vi "FuncVI-FileMove.vi"(5 "InstanceRef":T2, 9 "arg list":T1[](array[typedef]) {"num" format="%.2f"}) -> (0 "error out":bool, 3 "result":T1 {"num" format="%.2f"})   [LabVIEW 2021]
doc: "::: CalcExpress Toolkit :::\nCopyright (c) 2000-2026 Konstantin Shifershteyn. All rights reserved."
uses:
  cetypes.llb/CalcExpress Function Argument Info.ctl
  cetypes.llb/CalcExpress Instance RefNum.ctl
panel:
  in  "max arg num":i32=2
  in  "min arg num":i32=2
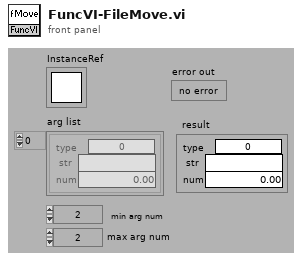
[diagram p1: front panel]
types:
  T1 = typedef "CalcExpress Function Argument Info.ctl" = cluster{"type":u32, "str":string, "num":dbl}
  T2 = typedef "CalcExpress Instance RefNum.ctl" = refnum<k1>
  T3 = enum32{"String", "DBL Number", "identifier", "1D Array of DBL", "2D Array of DBL", "CDB Number", "1D Array of CDB", "2D Array of CDB", "1D Array of String", "2D Array of String", "Unknown data type"}
  T4 = enum32{"existing file", "new file", "new or existing file", "existing dir", "new dir", "new or existing dir", "existing file (use LLBs)", "new file (use LLBs)", "new or existing file (use LLBs)", "new or existing file or directory (use LLBs)", "existing dir (use LLBs)", "new dir (use LLBs)", "new or existing dir (use LLBs)", "existing file or dir", "new file or dir", "new or existing file or dir", "existing file or dir (use LLBs)", "new file or dir (use LLBs)"}
  T5 = cluster{"type: use this constant to specify a predefined type code":enum32{"String", "DBL Number", "identifier", "1D Array of DBL", "2D Array of DBL", "CDB Number", "1D Array of CDB", "2D Array of CDB", "1D Array of String", "2D Array of String", "Unknown data type"}, string, "code":dbl}
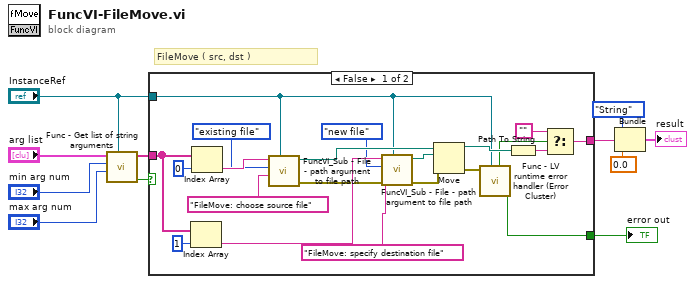
[diagram p0: block diagram]
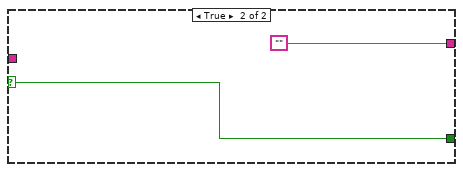
[diagram p2: hidden frame]
diagram:
  # "FileMove ( src, dst )"
  n1 = call "Func - Get list of string arguments.vi"("InstanceRef"="InstanceRef", "max arg num"="max arg num", "min arg num"="min arg num", "arg list"="arg list") -> ("error out"=w7:bool, "val list"=w8:string[])  [unwired: 4 in]
  n2 = case shown="False" w7 {
    selector: w7 -> [_ w34]
    tunnel: [w13 w34] -> w11
    tunnel: "InstanceRef" -> [w14 _]
    tunnel: w8 -> [w28 _]
    tunnel: [w16 ""] -> w3
    frame False {
      n3 = Index Array(array=w28, index=1) -> (element=w30:string)
      n4 = Index Array(array=w28, index=0) -> (element=w31:string)
      n5 = call "FuncVI_Sub - File - path argument to file path.vi"("InstanceRef"=w14, "prompt"="FileMove: choose source file", "select mode (2)"=T4."existing file", "arg: file path"=w31) -> ("error out"=w25:errorcluster, "file path"=w27:path)  [unwired: 5 in, 1 out]
      n6 = call "FuncVI_Sub - File - path argument to file path.vi"("InstanceRef"=w14, "error in"=w25, "prompt"="FileMove: specify destination file", "select mode (2)"=T4."new file", "arg: file path"=w30) -> ("error out"=w22:errorcluster, "file path"=w26:path)  [unwired: 4 in, 1 out]
      n7 = Move(source path=w27, error in=w22, 10:w26) -> (error out=w15:errorcluster, 3:w19:path)  [unwired: 2 in, 1 out]
      n8 = call "Func - LV runtime error handler (Error Cluster).vi"("InstanceRef"=w14, "LabVIEW error"=w15) -> ("error out"=w13:bool, "LV error status"=w12:bool)  [unwired: 4 in, 2 out]
      n9 = Path To String(path=w19) -> (string=w18:string)
      n10 = Select(t="", s=w12, f=w18) -> (s? t:f=w16:string)
    }
    frame True {
    }
  }
  "error out" <- w11
  n11 = Bundle("type: use this constant to specify a predefined type code"=T3."String", w3, "code"=0.0) -> (→"result":T5)  [unwired: 1 in]
